vi "PicoScope4000aExampleStreaming.vi"() -> ()   [LabVIEW 2016]
doc: "This example demonstrates how to use the PicoScope Labview library to stream data from a PicoScope 5000 Series Device"
uses:
  ps4000a.dll
  PicoScope4000aLib/PicoScope4000aAnalogChannelSettings.ctl
panel:
  in  "Trigger Settings":T1={"Trigger Enabled"=FALSE, "Trigger Source"=enum."Channel A", "Trigger Threshold (Volts/Probe units)"=0.0, "Trigger Direction"=2, "Trigger Delay (samples)"=0, "Auto Trigger Time (ms)"=1000} {"Trigger Direction" items=["Rising"=2, "Falling"=3]}
  out "Analog Channels":cluster{i32, dbl, "Data (Volts)":dbl[]}[](graph)=[{0, 8e-09, "Data (Volts)"=[]}, {0, 8e-09, "Data (Volts)"=[]}, {0, 8e-09, "Data (Volts)"=[]}, {0, 8e-09, "Data (Volts)"=[]}, {0, 8e-09, "Data (Volts)"=[]}, {0, 8e-09, "Data (Volts)"=[]}, {0, 8e-09, "Data (Volts)"=[]}, {0, 8e-09, "Data (Volts)"=[]}]
  in  "Channel B Settings":T2={"Enabled"=FALSE, "Coupling"=1, "Range"=6, "Analogue Offset"=0.0, "Bandwidth Limit"=0} {"Bandwidth Limit" items=["Full", "20kHz", "100kHz", "1MHz"]; "Range" items=["10 mV", "20 mV", "50 mV", "100 mV", "200 mV", "500 mV", "1 V", "2 V", "5 V", "10 V", "20 V", "50 V ", "100 V"]; "Coupling" items=["AC", "DC"]}
  in  "Channel A Settings":T2={"Enabled"=TRUE, "Coupling"=1, "Range"=6, "Analogue Offset"=0.0, "Bandwidth Limit"=0} {"Bandwidth Limit" items=["Full", "20kHz", "100kHz", "1MHz"]; "Range" items=["10 mV", "20 mV", "50 mV", "100 mV", "200 mV", "500 mV", "1 V", "2 V", "5 V", "10 V", "20 V", "50 V ", "100 V"]; "Coupling" items=["AC", "DC"]}
  out "Raw Sample Interval (sec)":dbl=1.0000000130088963e-06 format="%#.5p"
  out "Max ADC value":i16
  out "Chunk time":u32
  out "Elapsed time":dbl
  in  "Poll time (ms)":u32=10 min=1 max=1000 step=1
  in  "Data file":path=path "PicoScope4000aExampleStreaming ChA Data"
  out "size(s)":i32
  out "Queue depth":i32(graph)
  out "queue depth":i32
  in  "Buffer and Transfer Settings":T3={"startIndex"=0, "Samples"=1000000, "Down Sample Ratio"=1, "Down-Sample Mode"=0} {"Down-Sample Mode" items=["None"=0, "Aggregate"=1, "Decimate"=2, "Average"=4]; "Down Sample Ratio" step=1; "Samples" format="%_6p"}
  out "USB Powered":bool=TRUE
  out "USB 3.0 device on non-USB 3.0 Port":bool=TRUE
  out "TriggeredAt (In Buffer)":u32 format="%#.6p"
  out "TriggeredAt (Total samples)":u32 format="%#.6p"
  in  "Acquisition Settings":T4={"Auto Stop"=TRUE, "Desired Sample Interval"=1, "Pre-trigger Samples"=0, "Post-trigger Samples"=1000000, "Down-Sample Ratio"=1, "Down-Sample Mode"=0, "Time Units"=3} {"Time Units" items=["Nanoseconds (ns)"=2, "Microseconds (us)"=3, "Milliseconds (ms)"=4, "Seconds (s)"=5]; "Down-Sample Mode" items=["None"=0, "Aggregate"=1, "Decimate"=2, "Average"=4]; "Post-trigger Samples" format="%#.6p"; "Pre-trigger Samples" format="%#_6p"}
  out "Triggered":bool
  out "DownSample Interval (sec)":dbl=1.0000000130088963e-06 format="%#.5p"
  out "Total Samples":u32 format="%#.6p"
  out "Auto Stopped":bool
  in  "Serial Number":string
  in  "Open Using Serial Number":bool
  out "Number of Samples per Capture":u32 format="%#.6p"
  in  "Resolution":u32(ring)=1 items=["8-bit", "12-bit", "14-bit", "15-bit (max. 2 ch.)", "16-bit (max. 1 ch.)"]
  in  "Apply  Settings":bool
  in  "stop":bool
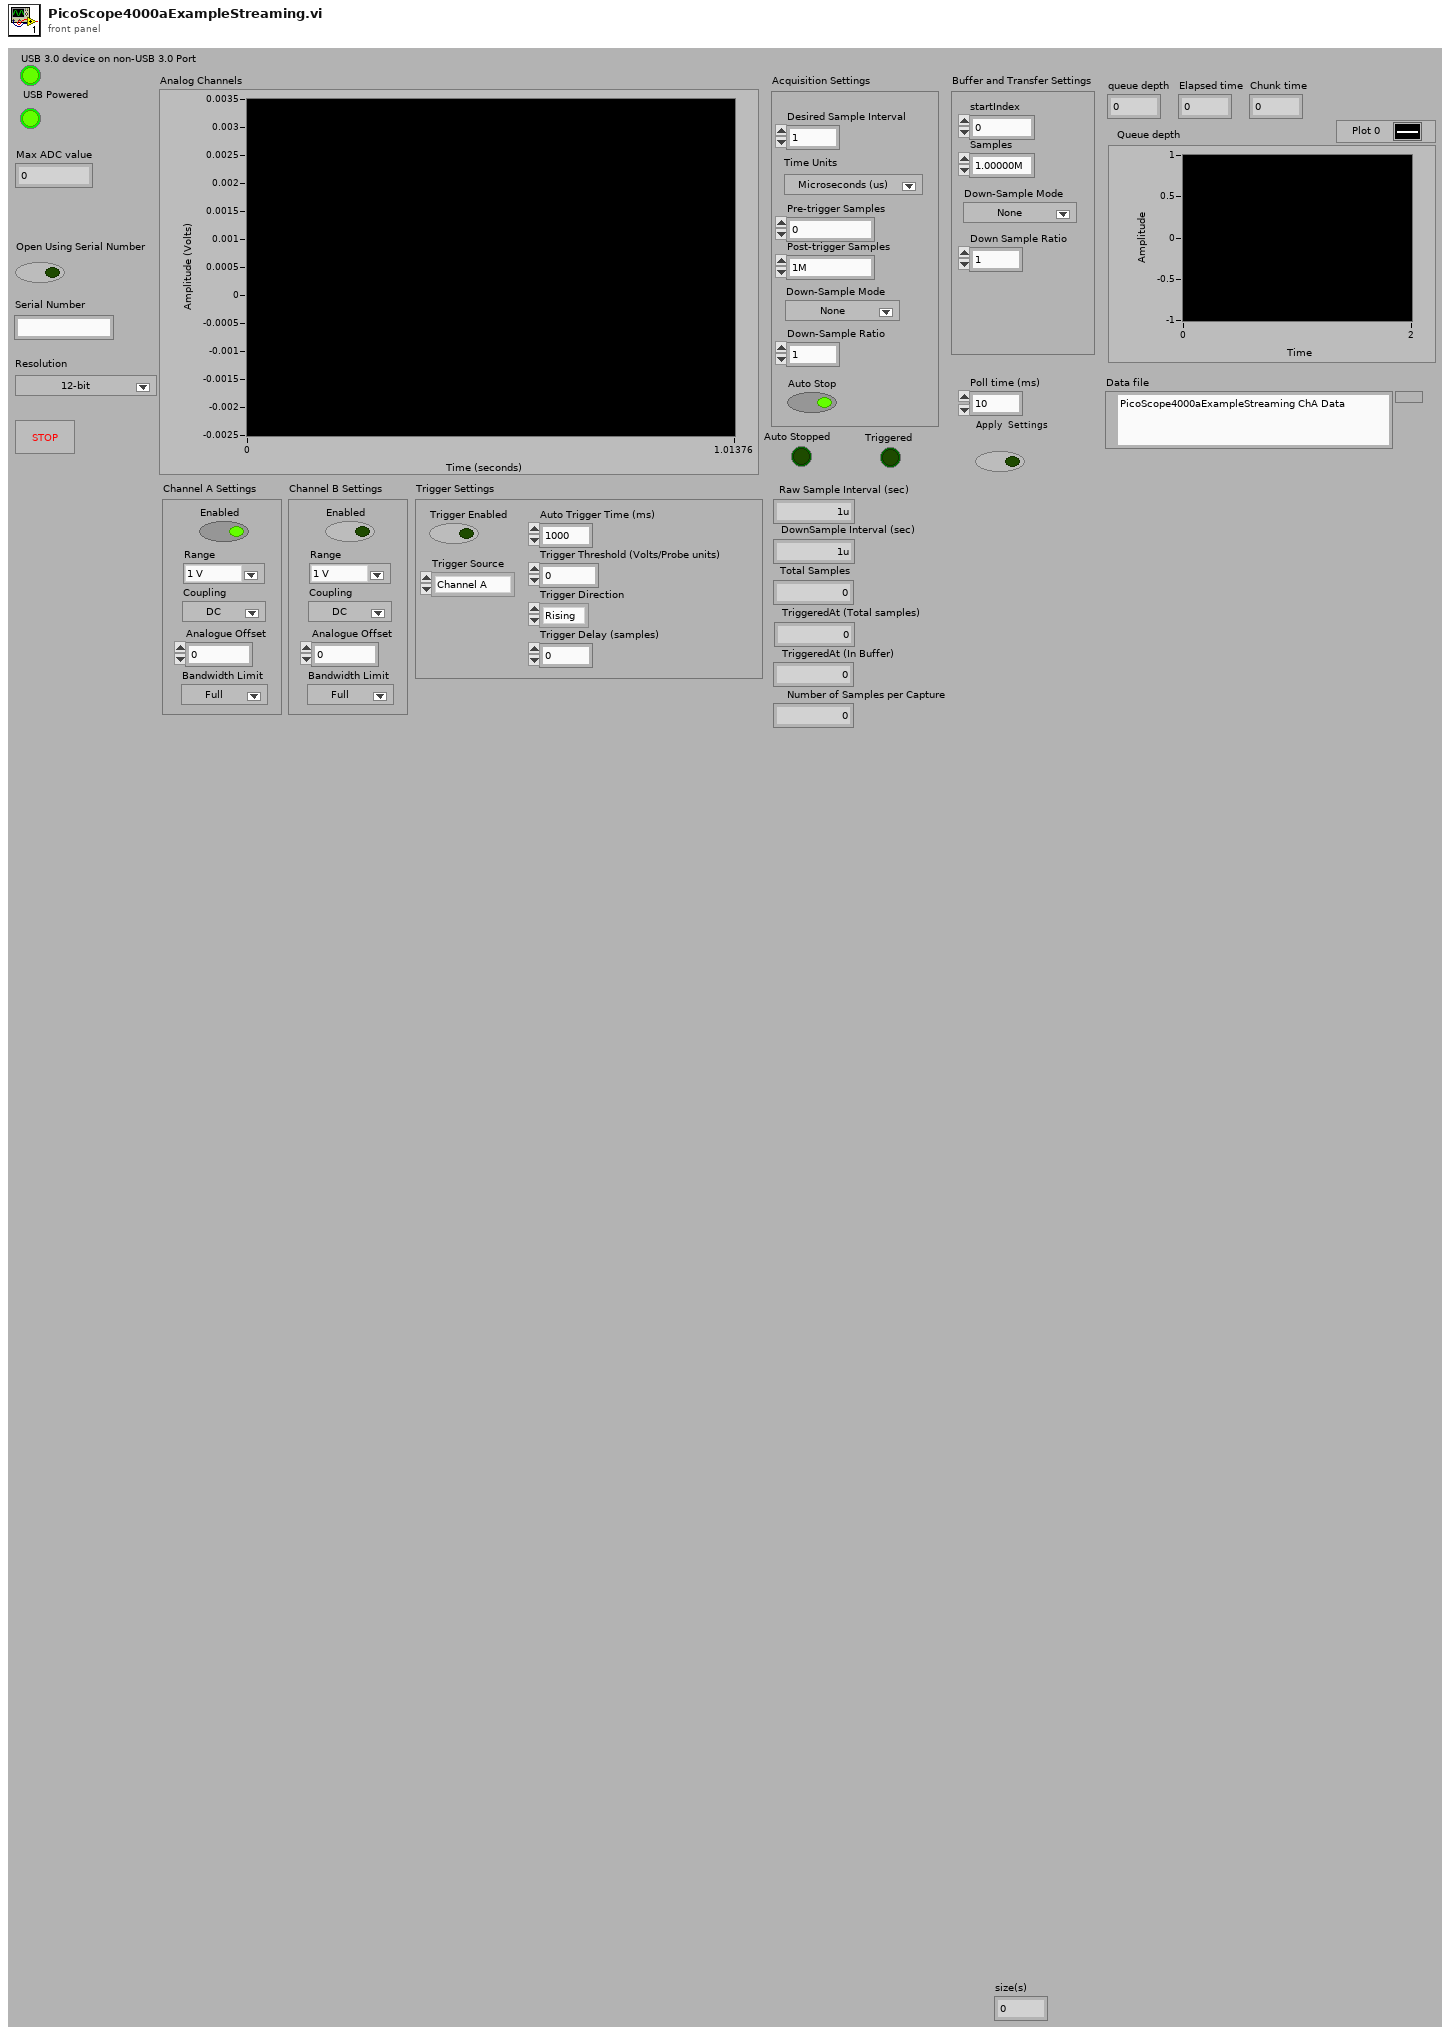
[diagram p1: front panel]
types:
  T1 = cluster{"Trigger Enabled":bool, "Trigger Source":enum16{"Channel A", "Channel B", "Channel C", "Channel D", "Channel E", "Channel F", "Channel G", "Channel H"}, "Trigger Threshold (Volts/Probe units)":dbl, "Trigger Direction":u16, "Trigger Delay (samples)":u32, "Auto Trigger Time (ms)":i16}
  T2 = typedef "PicoScope4000aAnalogChannelSettings.ctl" = cluster{"Enabled":bool, "Coupling":i16, "Range":u16, "Analogue Offset":sgl, "Bandwidth Limit":u32}
  T3 = cluster{"startIndex":u64, "Samples":u64, "Down Sample Ratio":u64, "Down-Sample Mode":u32}
  T4 = cluster{"Auto Stop":bool, "Desired Sample Interval":u32, "Pre-trigger Samples":u32, "Post-trigger Samples":u32, "Down-Sample Ratio":u32, "Down-Sample Mode":i32, "Time Units":u32}
  T5 = enum16{"open", "open or create", "create or replace", "create", "open (read-only)"}
  T6 = cluster{"Driver Version":string, "USB Version":string, "Hardware":string, "Variant":string, "Batch and Serial":string, "Cal Date":string, "Kernel Version":string, "Digital HW Version":string, "Analogue HW Version":string, "Firmware 1":string, "Firmware 2":string, "Num. channels":i16}
  T7 = cluster{i32, "DownSample Interval (sec)":dbl, "Data":dbl[]}
  T8 = cluster{i32, "DownSample Interval (sec)":dbl, "Data":dbl[]}[]
  T9 = cluster{"Channel A Buffer":i16[], "Channel B Buffer":i16[], "Channel C Buffer":i16[], "Channel D Buffer":i16[], "Channel E Buffer":i16[], "Channel F Buffer":i16[], "Channel G Buffer":i16[], "Channel H Buffer":i16[], "Port 0":i16[], "Port 1":i16[]}
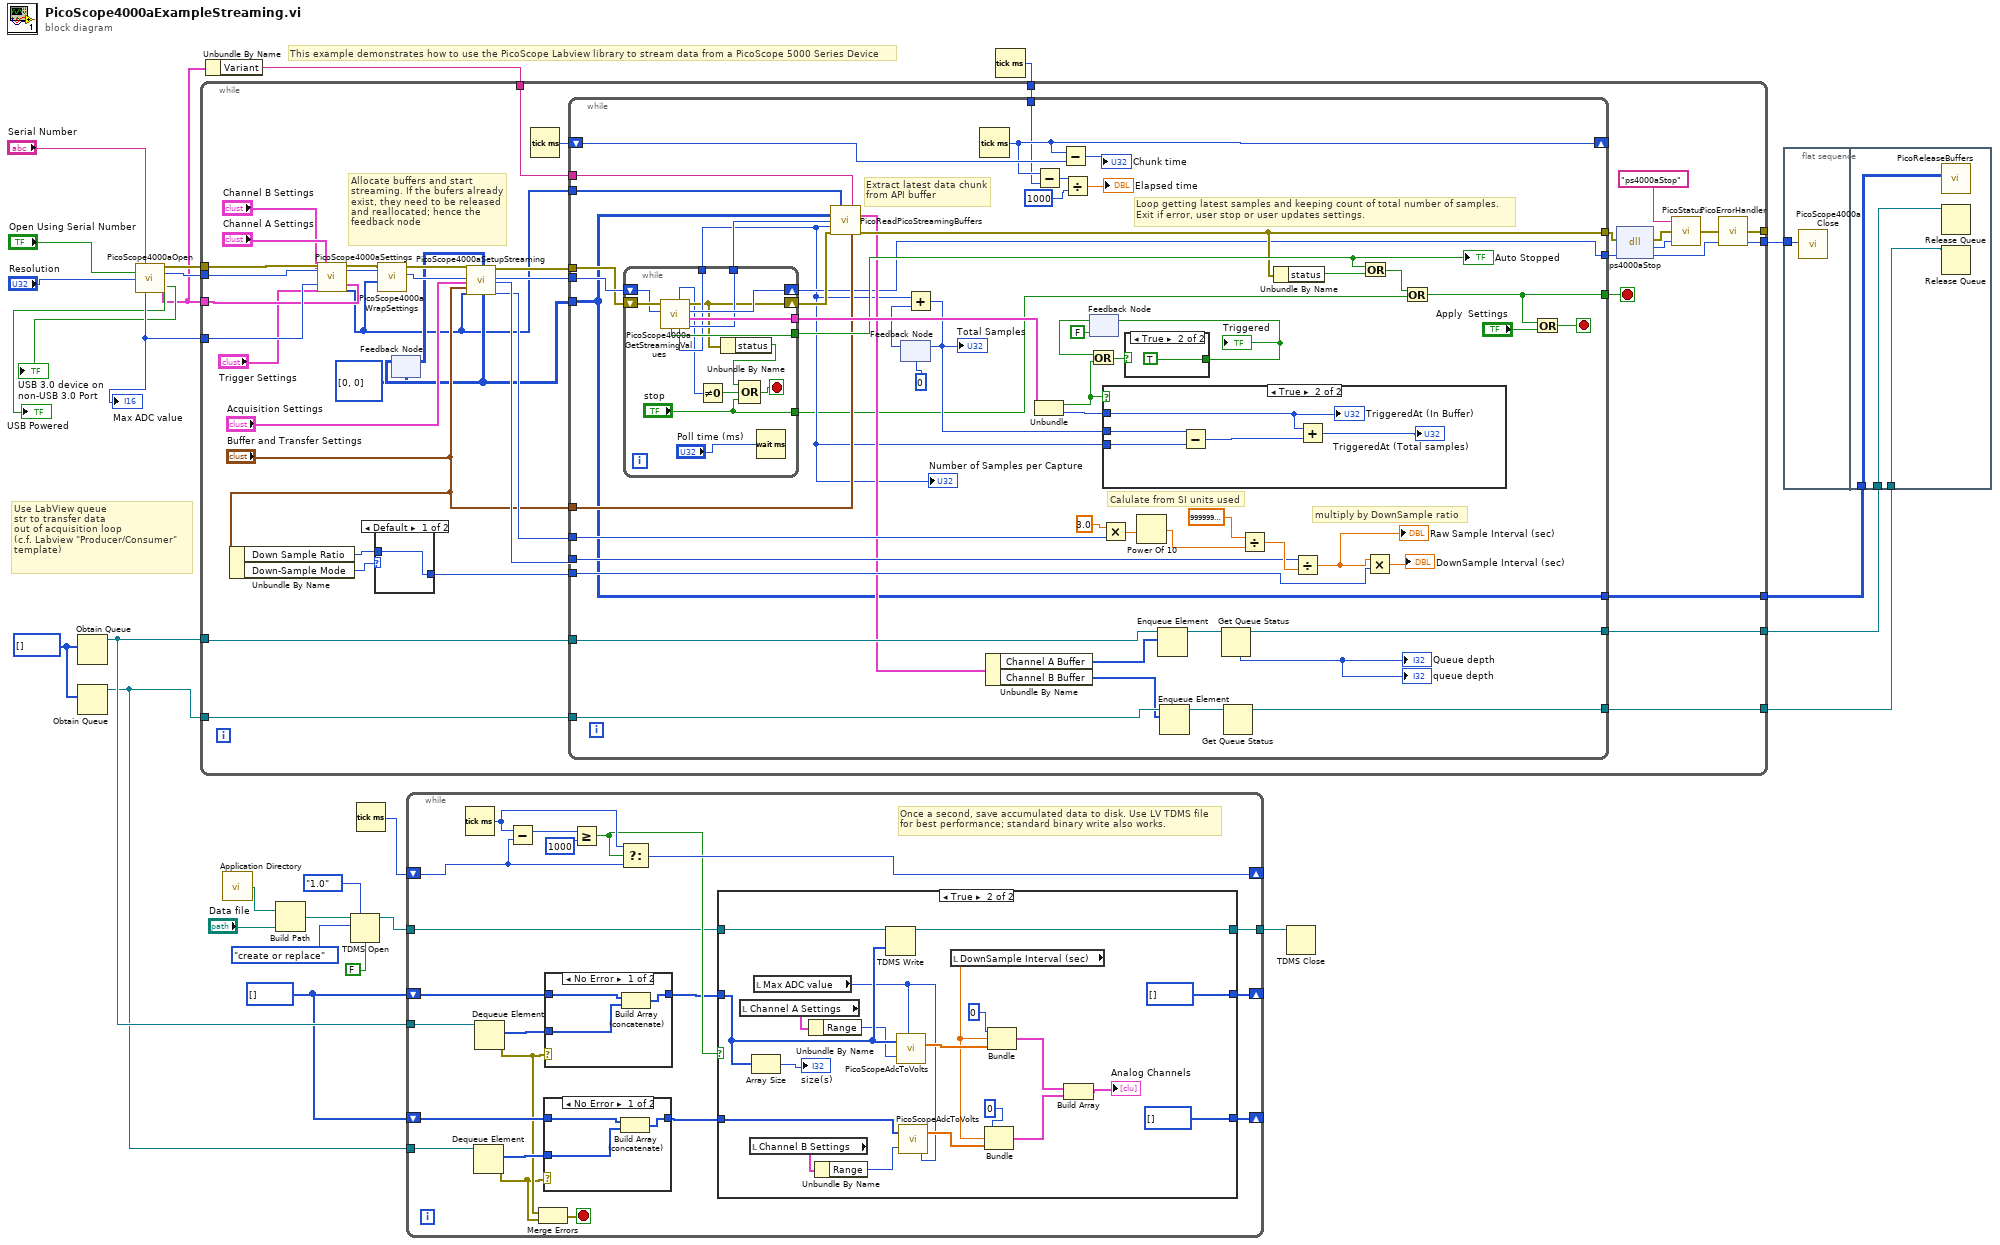
[diagram p0: block diagram]
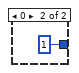
[diagram p5: hidden frame]
diagram:
  w6 = i16[] [] ("History Data")
  w9 = i16[] [] ("History Data")
  # "Use LabView queue\nstr to transfer data\nout of acquisition loop\n(c.f. Labview \"Producer/Consumer\"\ntemplate)"
  # "This example demonstrates how to use the PicoScope Labview library to stream data from a PicoScope 5000 Series Device"
  n1 = Obtain Queue(element data type=w9) -> (queue out=w22:refnum<queue>)  [unwired: 4 in, 2 out]
  n2 = Obtain Queue(element data type=w9) -> (queue out=w7:refnum<queue>)  [unwired: 4 in, 2 out]
  n3 = call "PicoScope4000aOpen.vi"("Serial Number"="Serial Number", "Use Serial Number"="Open Using Serial Number", "Resolution"="Resolution") -> ("error out"=w28:errorcluster, "handle"=w27:i16, "Unit Info"=w2:T6, "Max ADC value"=w23:i16, "USB powered"=→"USB 3.0 device on non-USB 3.0 Port":bool, "USB 3.0 on non-USB 3.0 port"=→"USB Powered":bool)  [unwired: 7 in]
  "Max ADC value" <- w23
  n4 = Unbundle By Name(w2) -> ("Variant"=w1:string)
  n5 = call <vilib>:"Application Directory.vi"() -> ("Application Directory"=w3:path)
  n6 = Build Path(base path=w3, name or relative path="Data file") -> (appended path=w4:path)
  n7 = TDMS Open(6:FALSE ("disable buffering? (T)"), 7:enum16{"1.0", "2.0"}."1.0" ("file format version (2.0)"), 10:T5."create or replace" ("operation (0:open)"), 11:w4) -> (3:w13:refnum<k34>)  [unwired: 3 in, 1 out]
  n8 = Tick Count (ms)() -> (millisecond timer value=w15:u32)
  n9 = while {
    tunnel: w22 -> [w48]
    shift-right: [w39] -> _
    shift-left: w6 -> [w47]
    shift-right: [w42] -> _
    shift-left: w15 -> [w43]
    tunnel: w13 -> [w38]
    tunnel: [w37] -> w12
    tunnel: w7 -> [w35]
    shift-right: [w32] -> _
    shift-left: w6 -> [w34]
    stop <- w31 stop-if-true
    # "Once a second, save accumulated data to disk. Use LV TDMS file\nfor best performance; standard binary write also works."
    n10 = Tick Count (ms)() -> (millisecond timer value=w44:u32)
    n11 = Dequeue Element(queue=w35) -> (element=w36:i16[], error out=w29:errorcluster)  [unwired: 2 in, 2 out]
    n12 = Dequeue Element(queue=w48) -> (element=w49:i16[], error out=w30:errorcluster)  [unwired: 2 in, 2 out]
    n13 = Subtract(x=w44, y=w43) -> (x-y=w46:u32)
    n14 = Merge Errors(w30, w29) -> (w31:errorcluster)
    n15 = case shown="No Error" w29 {
      tunnel: w34 -> [w52 w53]
      tunnel: [w51 w53] -> w33
      tunnel: w36 -> [w50 _]
      frame No Error {
        n16 = Build Array (concatenate)(w52, w50) -> (w51:i16[])
      }
      frame Error {
      }
    }
    n17 = case shown="No Error" w30 {
      tunnel: w47 -> [w79 w80]
      tunnel: [w78 w80] -> w40
      tunnel: w49 -> [w77 _]
      frame No Error {
        n18 = Build Array (concatenate)(w79, w77) -> (w78:i16[])
      }
      frame Error {
      }
    }
    n19 = Greater Or Equal?(x=w46, y=u32 1000) -> (x >= y?=w41:bool)
    n20 = Select(t=w44, s=w41, f=w43) -> (s? t:f=w42:u32)
    n21 = case shown="True" w41 {
      tunnel: w40 -> [w56 w72]
      tunnel: [w56 i16[] [] ("History Data")] -> w39
      tunnel: w38 -> [w55 w74]
      tunnel: [w55 w73] -> w37
      tunnel: w33 -> [w54 w60]
      tunnel: [w54 i16[] [] ("History Data")] -> w32
      frame False {
      }
      frame True {
        n22 = local read "Channel A Settings"() -> (w59:T2)
        n23 = local read "Channel B Settings"() -> (w58:T2)
        n24 = Array Size(array=w72) -> (size(s)=→"size(s)":i32)
        n25 = local read "Max ADC value"() -> (w62:i16)
        n26 = Unbundle By Name(w59) -> ("Range"=w71:u16)
        n27 = Unbundle By Name(w58) -> ("Range"=w61:u16)
        n28 = TDMS Write(0:w74, 9:w72) -> (4:w73:refnum<k34>)  [unwired: 4 in, 3 out]
        n29 = call "PicoScopeAdcToVolts.vi"("Max_adc"=w62, "Range Index"=w71, "Data"=w72) -> ("Data"=w69:dbl[])
        n30 = call "PicoScopeAdcToVolts.vi"("Max_adc"=w62, "Range Index"=w61, "Data"=w60) -> ("Data"=w67:dbl[])
        n31 = local read "DownSample Interval (sec)"() -> (w66:dbl)
        n32 = Bundle(0, "DownSample Interval (sec)"=w66, "Data"=w67) -> (w63:T7)  [unwired: 1 in]
        n33 = Bundle(0, "DownSample Interval (sec)"=w66, "Data"=w69) -> (w64:T7)  [unwired: 1 in]
        n34 = Build Array(w64, w63) -> (→"Analog Channels":T8)
      }
    }
  }
  n35 = Tick Count (ms)() -> (millisecond timer value=w21:u32)
  n36 = while {
    tunnel: [w115] -> w20
    tunnel: w28 -> [w119]
    tunnel: w27 -> [w120]
    tunnel: w2 -> [w85]
    tunnel: w23 -> [w103]
    tunnel: [w97] -> w18
    tunnel: w22 -> [w96]
    tunnel: [w95] -> w19
    tunnel: [w93] -> _
    tunnel: w21 -> [w91]
    tunnel: [w88] -> w8
    tunnel: w7 -> [w87]
    tunnel: w1 -> [w81]
    stop <- w121 stop-if-true
    # "Allocate buffers and start\nstreaming. If the bufers already\nexist, they need to be released\nand reallocated; hence the\nfeedback node"
    n37 = Unbundle By Name("Buffer and Transfer Settings") -> ("Down Sample Ratio"=w100:u64, "Down-Sample Mode"=w102:u32)
    n38 = call "PicoScope4000aSettings.vi"("error in"=w119, "handle in"=w120, "Max ADC value"=w103, "Trigger Settings"="Trigger Settings", "Channel A Settings"="Channel A Settings", "Channel B Settings"="Channel B Settings", "Unit Info"=w85) -> ("error out"=w108:errorcluster, "handle out"=w107:i16, "Enabled array"=w83:i16[])  [unwired: 10 in]
    n39 = case shown="Default" w102 {
      tunnel: [w122 u32 1 ("Down-Sample Ratio")] -> w101
      tunnel: w100 -> [w122 _]
      frame Default {
      }
      frame 0 {
      }
    }
    n40 = call "PicoScope4000aWrapSettings.vi"("Enabled array"=w83, "Handle In"=w107, "error in (no error)"=w108) -> ("Handle Out"=w110:i16, "error out"=w109:errorcluster)  [unwired: 7 in]
    n41 = feedback #1(u64[][] [[0], [0]] ("Pointer array")) -> (w94:u64[][])
    n42 = call "PicoScope4000aSetupStreaming.vi"("error in"=w109, "handle in"=w110, "Acquisition Settings"="Acquisition Settings", "Buffer and Transfer Settings"="Buffer and Transfer Settings", "enabled array"=w83, "Pointers In"=w94) -> ("Pointer array"=w90:u64[][], "error out"=w117:errorcluster, "handle out"=w118:i16, "Sample Interval"=w106:u32, "sampleIntervalTimeUnits"=w105:u32)  [unwired: 9 in]
    n43 = feedback-in #1(w90) -> ()
    n44 = Tick Count (ms)() -> (millisecond timer value=w92:u32)
    n45 = while {
      tunnel: [w134] -> w116
      tunnel: [w177] -> w121
      tunnel: w118 -> [w153]
      tunnel: w117 -> [w152]
      tunnel: w106 -> [w156]
      tunnel: w105 -> [w164]
      tunnel: [w149] -> w104
      tunnel: w101 -> [w154]
      tunnel: "Buffer and Transfer Settings" -> [w151]
      tunnel: w83 -> [w148]
      tunnel: [w146] -> w97
      tunnel: w96 -> [w144]
      tunnel: w90 -> [w142]
      tunnel: [w142] -> w95
      shift-right: [w137] -> _
      shift-left: w92 -> [w138]
      tunnel: w91 -> [w136]
      tunnel: w81 -> [w130]
      tunnel: [w127] -> w88
      tunnel: w87 -> [w126]
      stop <- w176 stop-if-true
      # "Loop getting latest samples and keeping count of total number of samples. \nExit if error, user stop or user updates settings."
      # "Extract latest data chunk\nfrom API buffer"
      # "Calulate from SI units used"
      # "multiply by DownSample ratio"
      n46 = while {
        tunnel: [w192] -> w175
        tunnel: [w191] -> w172
        tunnel: [w188] -> w132
        tunnel: [w187] -> w131
        shift-right: [w189] -> w134
        shift-left: w153 -> [w179]
        shift-right: [w186] -> w150
        shift-left: w152 -> [w190]
        tunnel: ["stop"] -> w124
        stop <- w181 stop-if-true
        n47 = call "PicoScope4000aGetStreamingValues.vi"("handle in"=w179, "error in"=w190) -> ("Start Index in Driver Buffer"=w188:u32, "Trigger"=w192:cluster{bool, "triggeredAt (Total samples)":u32}, "handle out"=w189:i16, "error out"=w186:errorcluster, "Number of Samples"=w187:u32, "ready"=w184:i16, "Auto Stopped"=w191:bool)  [unwired: 3 in]
        n48 = Not Equal To 0?(x=w184) -> (x != 0?=w182:bool)
        n49 = Unbundle By Name(w186) -> ("status"=w183:bool)
        n50 = Compound Arithmetic op=OR(w183, w182, "stop") -> (w181:bool)
        n51 = Wait (ms)(milliseconds to wait="Poll time (ms)") -> ()  [unwired: 1 out]
      }
      "Number of Samples per Capture" <- w131
      "Auto Stopped" <- w172
      n52 = call "PicoReadPicoStreamingBuffers.vi"("enabled array"=w148, "Buffer and Transfer Settings"=w151, "Variant"=w130, "Pointer array"=w142, "Offset Index"=w132, "Number of Samples"=w131, "error in (no error)"=w150) -> ("Buffers (Max or non-aggregated)"=w143:T9, "error out"=w149:errorcluster)  [unwired: 7 in]
      n53 = feedback #2(u32 0) -> (w168:u32)
      n54 = Add(x=w131, y=w168) -> (x+y=w160:u32)
      "Total Samples" <- w160
      n55 = feedback-in #2(w160) -> ()
      n56 = Tick Count (ms)() -> (millisecond timer value=w137:u32)
      n57 = Unbundle By Name(w143) -> ("Channel A Buffer"=w133:i16[], "Channel B Buffer"=w125:i16[])
      n58 = Subtract(x=w137, y=w136) -> (x-y=w141:u32)
      n59 = Unbundle(w175) -> (w158:bool, "triggeredAt (Total samples)"=w157:u32)
      n60 = Subtract(x=w137, y=w138) -> (x-y=→"Chunk time":u32)
      n61 = Divide(x=w141, y=u32 1000) -> (x/y=→"Elapsed time":dbl)
      n62 = feedback #3(FALSE) -> (w170:bool)
      n63 = Or(x=w170, y=w158) -> (x .or. y?=w161:bool)
      n64 = Multiply(x=3.0, y=w164) -> (x*y=w162:dbl)
      n65 = case shown="True" w158 {
        tunnel: w131 -> [_ w193]
        tunnel: w160 -> [_ w197]
        tunnel: w157 -> [_ w195]
        frame False {
        }
        frame True {
          n66 = Subtract(x=w197, y=w193) -> (x-y=w196:u32)
          n67 = Add(x=w195, y=w196) -> (x+y=→"TriggeredAt (Total samples)":u32)
          "TriggeredAt (In Buffer)" <- w195
        }
      }
      n68 = case shown="True" w161 {
        selector: w161 -> [w198 _]
        tunnel: [w198 TRUE] -> w159
        frame False {
        }
        frame True {
        }
      }
      "Triggered" <- w159
      n69 = feedback-in #3(w159) -> ()
      n70 = Power Of 10(x=w162) -> (10^x=w163:dbl)
      n71 = Enqueue Element(queue=w144, element=w133) -> (queue out=w145:refnum<queue>)  [unwired: 2 in, 2 out]
      n72 = Enqueue Element(queue=w126, element=w125) -> (queue out=w128:refnum<queue>)  [unwired: 2 in, 2 out]
      n73 = Get Queue Status(queue=w145) -> (queue out=w146:refnum<queue>, # elements in queue=→"queue depth" →"Queue depth":i32)  [unwired: 2 in, 6 out]
      n74 = Get Queue Status(queue=w128) -> (queue out=w127:refnum<queue>)  [unwired: 2 in, 7 out]
      n75 = Divide(x=sgl 1000000000000000.0 ("y"), y=w163) -> (x/y=w165:dbl)
      n76 = Unbundle By Name(w149) -> ("status"=w174:bool)
      n77 = Divide(x=w156, y=w165) -> (x/y=w129:dbl)
      "Raw Sample Interval (sec)" <- w129
      n78 = Or(x=w172, y=w174) -> (x .or. y?=w173:bool)
      n79 = Multiply(x=w129, y=w154) -> (x*y=→"DownSample Interval (sec)":dbl)
      n80 = Or(x=w173, y=w124) -> (x .or. y?=w177:bool)
      n81 = Or(x=w177, y="Apply  Settings") -> (x .or. y?=w176:bool)
    }
    n82 = dll-call lib="ps4000a.dll" fn="ps4000aStop"(error in=w104, "handle"=w116) -> (error out=w113:errorcluster, "PICO_STATUS"=w114:u32, "handle"=w115:i16)  [unwired: 2 in, 1 out]
    n83 = call "PicoStatus.vi"("PICO STATUS"=w114, "error in"=w113, "source"="ps4000aStop") -> ("error out"=w112:errorcluster)
    n84 = call "PicoErrorHandler.vi"("error in"=w112) -> ("error out"=w93:errorcluster)
  }
  n85 = TDMS Close(11:w12) -> ()  [unwired: 1 in, 2 out]
  n86 = flat-sequence {
    tunnel: w20 -> [w200]
    tunnel: w19 -> [w203]
    tunnel: w18 -> [w202]
    tunnel: w8 -> [w201]
    frame #0 {
      n87 = call "PicoScope4000aClose.vi"("handle"=w200) -> ()
    }
    frame #1 {
      n88 = call "PicoReleaseBuffers.vi"("Pointer array"=w203) -> ()  [unwired: 10 in, 1 out]
      n89 = Release Queue(queue=w202) -> ()  [unwired: 2 in, 3 out]
      n90 = Release Queue(queue=w201) -> ()  [unwired: 2 in, 3 out]
    }
  }
